vi "VIH Project Tree - Find Parent Group of an Item.vi"(8 "error in":errorcluster, 10 "Tree Item Tag":string, 11 "Project Tree":T1) -> (0 "error out":errorcluster, 1 "Level":i32, 2 "Parent Group Tag":string, 3 "dup Project Tree":T1)   [LabVIEW 2014]
doc: "::: VI Helpeks :::\nCopyright (c) 2000-2026 Konstantin Shifershteyn. All rights reserved."
uses:
  VIH Project Tree Typedef - Tree Refnum.ctl
panel:
  # "VI Helpeks\nCopyright (c) 2012-2026 Konstantin Shifershteyn"
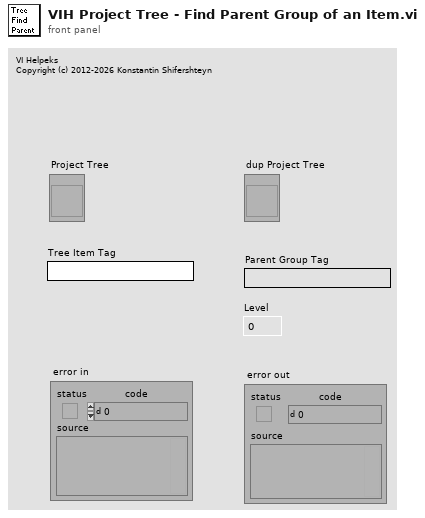
[diagram p1: front panel]
types:
  T1 = typedef "VIH Project Tree Typedef - Tree Refnum.ctl" = refnum<vi>
  T2 = typedef "VIH Project Tree Typedef - Tree Item Type.ctl" = enum32{"<Invalid>", "Project", "Proj Files", "Proj Rules", "File Group", "Rule Group", "Any File", "LV Func", ".mnu", ".mnu (dyn)", ".vi", ".vi (dyn)", ".vit", ".vit (dyn)", ".ctl", ".ctl (dyn)", ".ctt", ".ctt (dyn)", "polyVI", "polyVI (dyn)", "expVI", "expVI (dyn)", "HTML", "PolyVI Inst"}
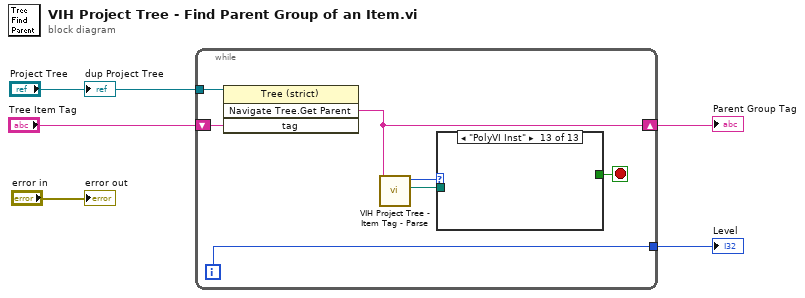
[diagram p0: block diagram]
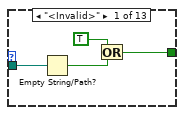
[diagram p2: hidden frame]
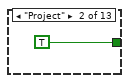
[diagram p3: hidden frame]
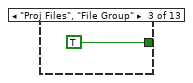
[diagram p4: hidden frame]
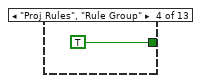
[diagram p5: hidden frame]
diagram:
  n1 = while {
    tunnel: "Project Tree" -> [w12]
    shift-right: [w9] -> w2
    shift-left: "Tree Item Tag" -> [w11]
    tunnel: [w7] -> w1
    i -> [w7]
    stop <- w8 stop-if-true
    n2 = invoke class="Tree (strict)" method="Navigate Tree.Get Parent"(reference=w12, "tag"=w11) -> ("Navigate Tree:Get Parent"=w9:string)  [unwired: 2 in, 3 out]
    n3 = call "VIH Project Tree - Item Tag - Parse.vi"("Tree Item Tag"=w9) -> ("Item File Path"=w6:path, "Item Type"=w10:T2)  [unwired: 8 in, 1 out]
    n4 = case shown="\"PolyVI Inst\"" w10 {
      tunnel: [w15 TRUE TRUE TRUE _ _ _ _ _ _ _ _ _] -> w8
      tunnel: w6 -> [w16 _ _ _ _ _ _ _ _ _ _ _ _]
      frame "<Invalid>" {
        n5 = Empty String/Path?(string/path=w16) -> (empty?=w13:bool)
        n6 = Or(x=TRUE, y=w13) -> (x .or. y?=w15:bool)
      }
      frame "Project" {
      }
      frame "Proj Files", "File Group" {
      }
      frame "Proj Rules", "Rule Group" {
      }
      frame "Any File" {
      }
      frame "LV Func" {
      }
      frame ".mnu", ".mnu (dyn)" {
      }
      frame ".vi"..".vit (dyn)" {
      }
      frame ".ctl"..".ctt (dyn)" {
      }
      frame "polyVI", "polyVI (dyn)" {
      }
      frame "expVI", "expVI (dyn)" {
      }
      frame "HTML" {
      }
      frame "PolyVI Inst" {
      }
    }
  }
  "Parent Group Tag" <- w2
  "Level" <- w1
  "error out" <- "error in"
  "dup Project Tree" <- "Project Tree"
